vi "UNITTEST-JSON-RPC-string-Element.vi"(8 "error in (no error)":errorcluster) -> (0 "error out":errorcluster)   [LabVIEW 2019]
uses:
  4c12f335-3af6-49f5-9257-0130b4f6318c.vi
  e861ad0b-bed5-4796-b07d-8449c8f87c08.vi
  JSON-RPC/API/JSON to Variant.vi
  <vilib>/Utility/Data Type/Get Type Information.vi
  <vilib>/JDP Science/JSONtext/JSON type.vi
  <vilib>/JDP Science/JSONtext/Get Array Elements.vi
  <vilib>/JDP Science/JSONtext/JSON text to Variant.vi
  <vilib>/addons/_JKI Toolkits/Caraya/classes/Assert/Assert Equal Value_Variant.vi
  <vilib>/addons/_JKI Toolkits/Caraya/classes/Assert/Assert Not Error.vi
  JSON-RPC/JSON-RPC.lvlib
  <vilib>/addons/_JKI Toolkits/Caraya/classes/Assert/Assert.lvclass
  <vilib>/addons/_JKI Toolkits/Caraya/classes/Test/Test.lvclass
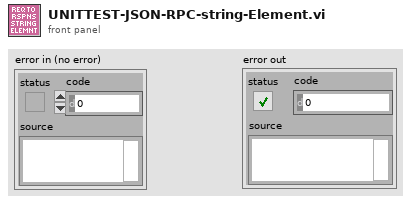
[diagram p1: front panel]
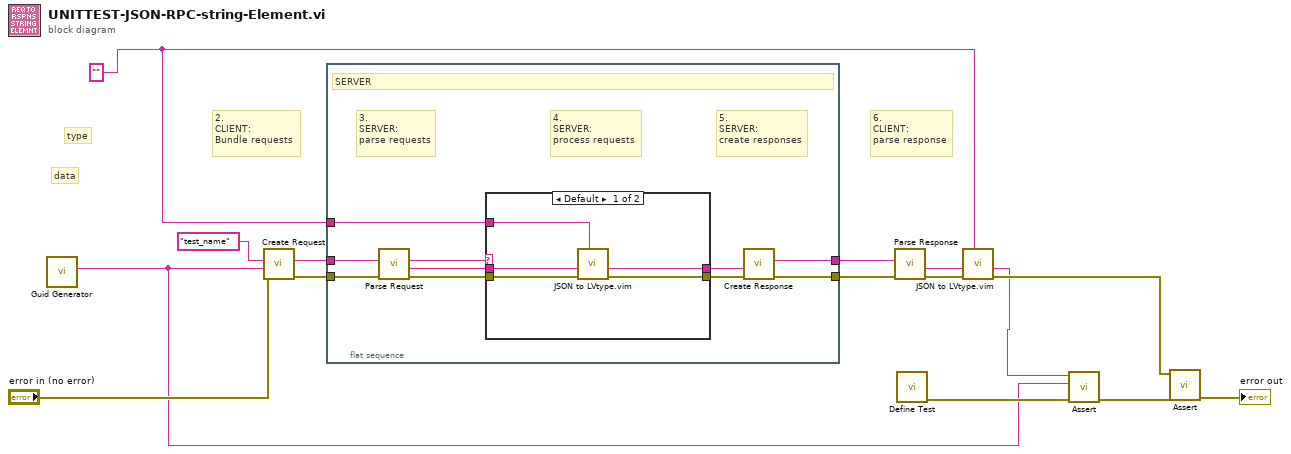
[diagram p0: block diagram]
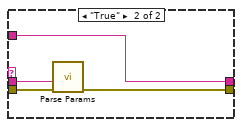
[diagram p2: hidden frame]
diagram:
  w1 = ""
  # "data"
  # "type"
  # "6.\nCLIENT:\nparse response"
  # "2.\nCLIENT:\nBundle requests"
  n1 = call <vilib>:"Guid Generator.vi"() -> ("GUID"=w2:string)  [unwired: 10 in, 1 out]
  n2 = call "Create Request.vi"("error in (no error)"="error in (no error)", "params"=w2, "method"="test_name") -> ("error out"=w14:errorcluster, "<JSON> Requests"=w15:string)  [unwired: 6 in, 1 out]
  n3 = flat-sequence {
    tunnel: w15 -> [w25]
    tunnel: w14 -> [w21]
    tunnel: [w20] -> w13
    tunnel: [w19] -> w12
    tunnel: w1 -> [w17]
    frame #0 {
      # "3.\nSERVER:\nparse requests"
      # "4.\nSERVER:\nprocess requests"
      # "5.\nSERVER:\ncreate responses"
      # "SERVER"
      n4 = call "Parse Request.vi"("error in (no error)"=w21, "<JSON> Requests"=w25) -> ("error out"=w22:errorcluster, "Params"=w23:string, "Methods"=w24:string)  [unwired: 6 in, 1 out]
      n5 = case shown="Default" w24 {
        tunnel: w23 -> [w27 w34]
        tunnel: w22 -> [w30 w33]
        tunnel: [w29 w32] -> w18
        tunnel: w17 -> [w28 w31]
        tunnel: [w26 w31] -> w16
        frame Default {
          n6 = call "JSON to LVtype.vim"("type"=w28, "error in (no error)"=w30, "JSON Data in"=w27) -> ("error out"=w29:errorcluster, "Data out"=w26:string)  [unwired: 7 in]
        }
        frame "True" {
          n7 = call "Parse Params.vi"("error in (no error)"=w33, "<JSON> Params"=w34) -> ("error out"=w32:errorcluster)  [unwired: 7 in, 2 out]
        }
      }
      n8 = call "Create Response.vi"("error in (no error)"=w18, "result"=w16) -> ("error out"=w19:errorcluster, "<JSON> Response"=w20:string)  [unwired: 8 in]
    }
  }
  n9 = call "Parse Response.vi"("error in (no error)"=w12, "<JSON> Response"=w13) -> ("error out"=w11:errorcluster, "results"=w4:string)  [unwired: 7 in, 1 out]
  n10 = call <vilib>:"Define Test.vi"() -> ("error out"=w7:errorcluster)  [unwired: 10 in, 1 out]
  n11 = call "JSON to LVtype.vim"("type"=w1, "error in (no error)"=w11, "JSON Data in"=w4) -> ("error out"=w9:errorcluster, "Data out"=w3:string)  [unwired: 7 in]
  n12 = call-poly <vilib>:"Assert.vi"("error in (no error)"=w7, "Actual"=w2, "Expected"=w3) -> ("error out"=w10:errorcluster)  [unwired: 7 in, 1 out]
  n13 = call-poly <vilib>:"Assert.vi"("error in (no error)"=w10, "Not Error?"=w9) -> ("error out"=→"error out":errorcluster)  [unwired: 8 in, 1 out]
